vi "Configuration Tool Main.vi"() -> ()   [LabVIEW 2014, in "Advanced Configuration Tool.lvlib"]
doc: "This is the main VI for the configuration editor."
uses:
  Advanced Configuration Tool.lvlib
  Controls/StateCluster.ctl
  Configuration Framework/Repository/NISE_CEF_Repository.lvclass
  Configuration Framework/Node/NodeRef.ctl
  Configuration Framework/Node/NISE_CEF_Node.lvclass
  Configuration Framework/Node/StandardEvents.ctl
  Configuration Framework/Node/UserEventRef.ctl
  Configuration Framework/Controls/EventCluster.ctl
  Configuration Framework/Node/NodeChangeEvent.ctl
  Configuration Framework/Node/CacheState.ctl
  Configuration Framework/Node/RefreshUIEvent.ctl
  Configuration Framework/Node/StopEvent.ctl
  Configuration Framework/glyph manager/glyph manager.ctl
  <vilib>/picture/picture.llb/imagedata.ctl
  <vilib>/Utility/error.llb/DialogType.ctl
  Classes/cRIO node/cRIO  node root.lvclass
  Configuration Framework/hierarchy repo/NISE_CEF_HierarchyRepo.lvclass
  Controls/AddMessage.ctl
  Controls/MoveMessage.ctl
  <vilib>/NI/AMC/Read Termination Message.vi
  <vilib>/NI/AMC/Create Single Message.vi
  <vilib>/NI/AMC/Update Message Routing Info.vi
  <vilib>/NI/AMC/Globals.vi
  <vilib>/NI/AMC/Send Message.vi
  <vilib>/NI/AMC/AMC.lvlib
  Configuration Framework/NISE_CEF_TreeControl.lvlib
  Configuration Framework/serializable configuration/NISE_CEF_serializable configuration.lvclass
  Configuration Framework/glyph manager/glyph manager.lvlib
panel:
  in  "View":string(tree)
  in  "Exit":bool
  # "Configurator"
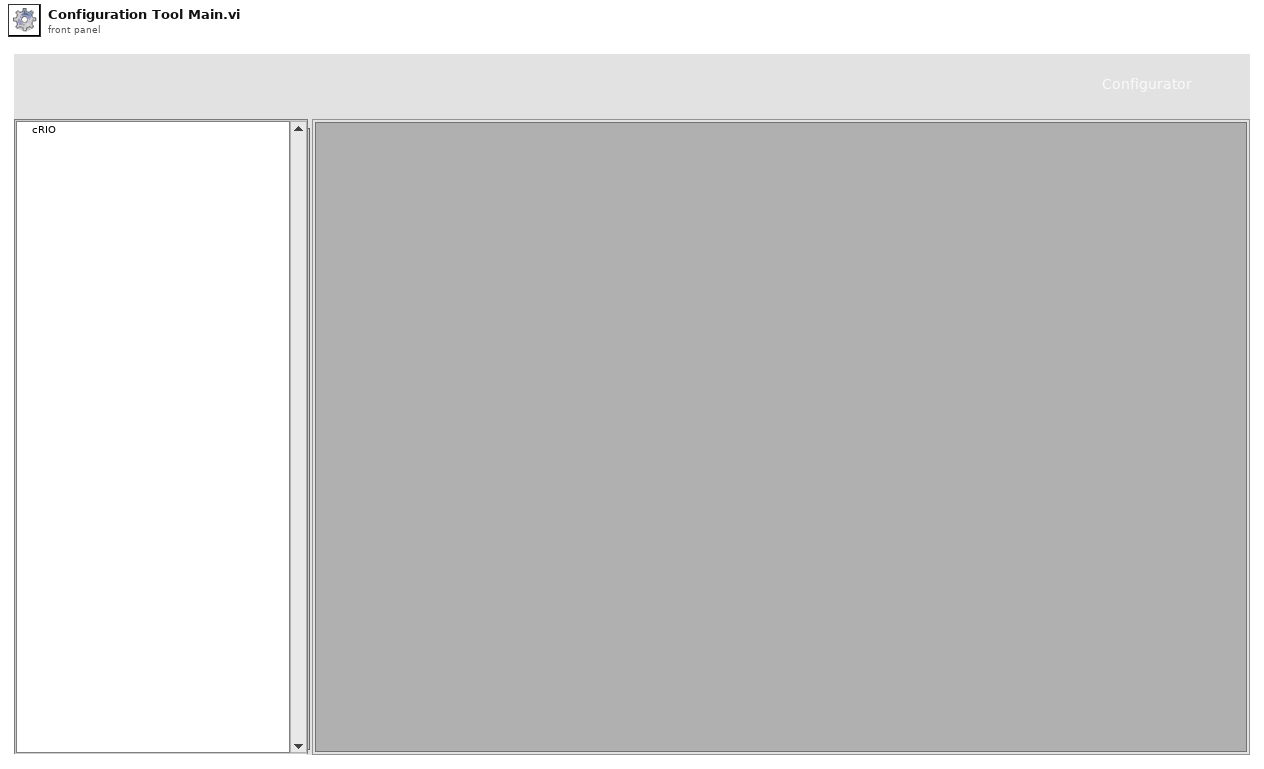
[diagram p1: front panel]
types:
  T1 = typedef "Advanced Configuration Tool.lvlib/StateCluster.ctl" = cluster{"repository":refnum<class "NISE_CEF_Repository.lvclass">, "root":T2, "unsaved changes":bool, "current path":path, "classes path":path, "standard events":T3, "glyph manager":T9}
  T2 = typedef "NISE_CEF_Node.lvclass/NodeRef.ctl" = refnum<data-value>
  T3 = typedef "NISE_CEF_Node.lvclass/StandardEvents.ctl" = cluster{"user event":T4, "node change":T5, "cache state":T6, "refresh UI":T7, "stop event":T8}
  T4 = typedef "NISE_CEF_Node.lvclass/UserEventRef.ctl" = refnum<user-event>
  T5 = typedef "NISE_CEF_Node.lvclass/NodeChangeEvent.ctl" = refnum<user-event>
  T6 = typedef "NISE_CEF_Node.lvclass/CacheState.ctl" = refnum<user-event>
  T7 = typedef "NISE_CEF_Node.lvclass/RefreshUIEvent.ctl" = refnum<user-event>
  T8 = typedef "NISE_CEF_Node.lvclass/StopEvent.ctl" = refnum<user-event>
  T9 = typedef "glyph manager.lvlib/glyph manager.ctl" = cluster{"search paths":path[], "glyph map":variant, "base glyphs":T10[], "desired overlays":string[]}
  T10 = typedef "imagedata.ctl" = cluster{"image type":i32, "image depth":i32, "image":u8[], "mask":u8[], "colors":u32[], "Rectangle":cluster{"left":i16, "top":i16, "right":i16, "bottom":i16}}
  T11 = typedef "AMC.lvlib/Message Queue.ctl" = refnum<queue>
  T12 = typedef "Advanced Configuration Tool.lvlib/AddMessage.ctl" = cluster{"node type":string, "to add to":string}
  T13 = typedef "Advanced Configuration Tool.lvlib/MoveMessage.ctl" = cluster{"node ref":T2, "new parent":T2, "Index":i32}
  T14 = typedef "Advanced Configuration Tool.lvlib/FilePaths.ctl" = cluster{"glyphs":path, "classes":path}
  T15 = typedef "DialogType.ctl" = u16
  T16 = typedef "NISE_CEF_Node.lvclass/Summary.ctl" = cluster{"ID":string, "parent ID":string, "node type":string, "text":string, "additional text":string, "glyph":string, "depth":i32, "glyph overlay":string}
  T17 = typedef "LVPoint32TypeDef.ctl" = cluster{"Horizontal":i32, "Vertical":i32}
  T18 = cluster{"data name":string, "drag data":variant}[]
  T19 = typedef "NISE_CEF_Node.lvclass/NodeMenuOptions.ctl" = cluster{"removable":bool, "movable":bool, "duplicate":bool}
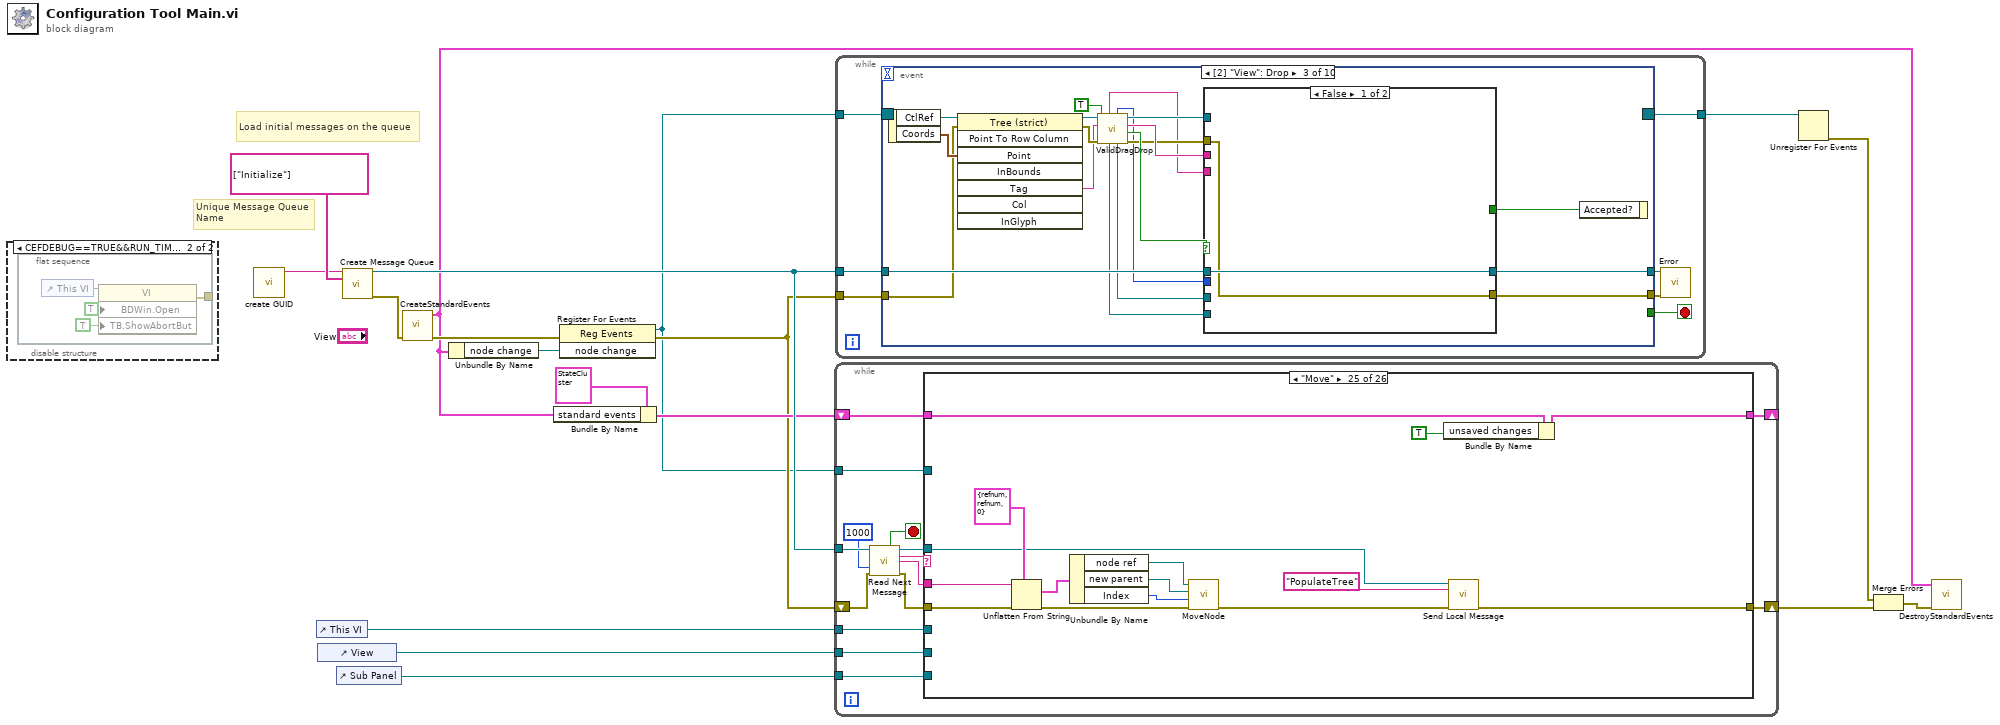
[diagram p0: block diagram]
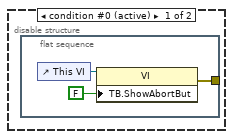
[diagram p2: hidden frame]
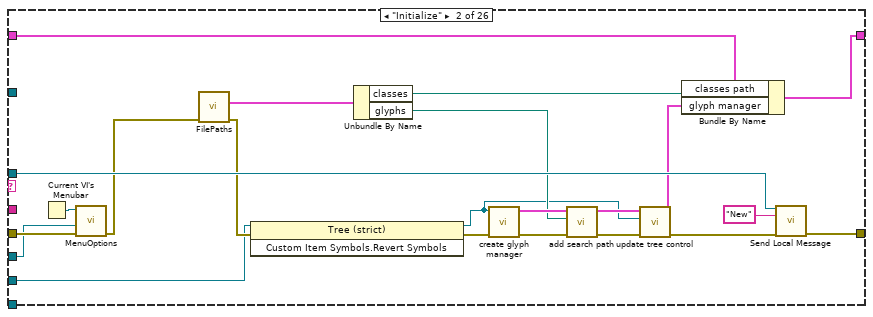
[diagram p4: hidden frame]
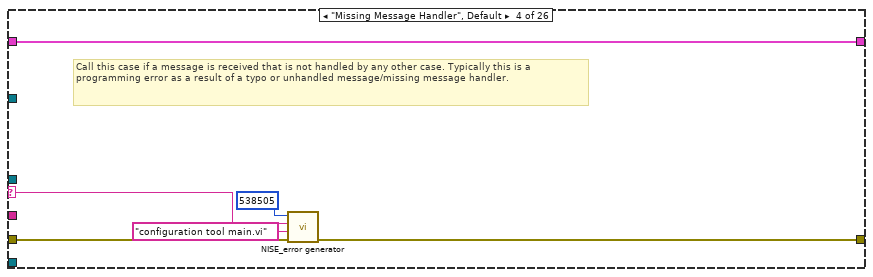
[diagram p6: hidden frame]
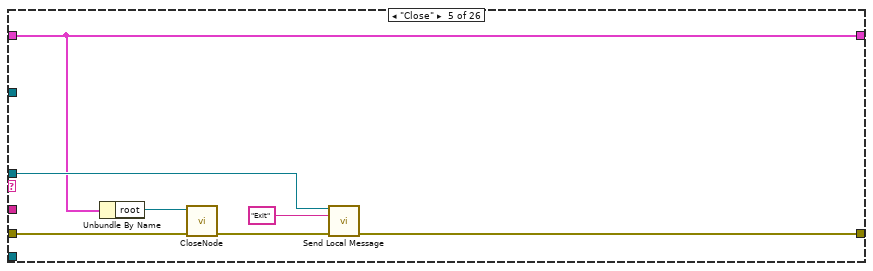
[diagram p7: hidden frame]
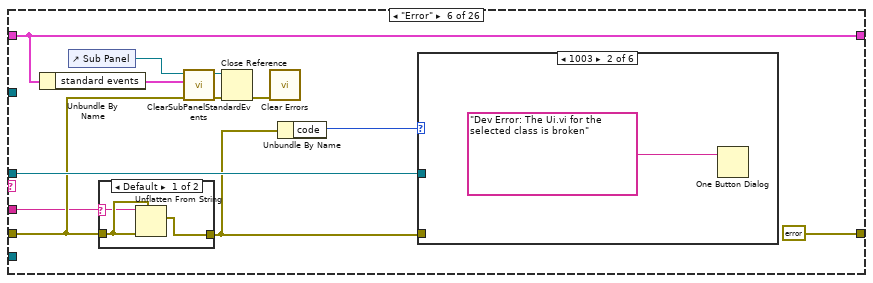
[diagram p8: hidden frame]
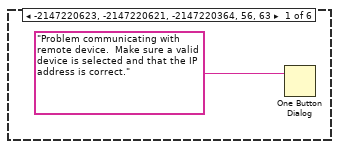
[diagram p10: hidden frame]
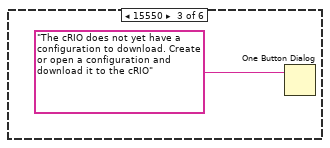
[diagram p11: hidden frame]
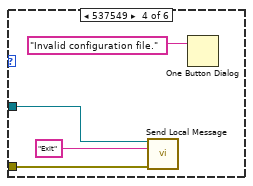
[diagram p12: hidden frame]
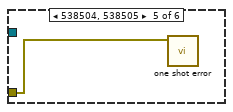
[diagram p13: hidden frame]
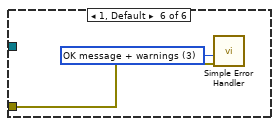
[diagram p14: hidden frame]
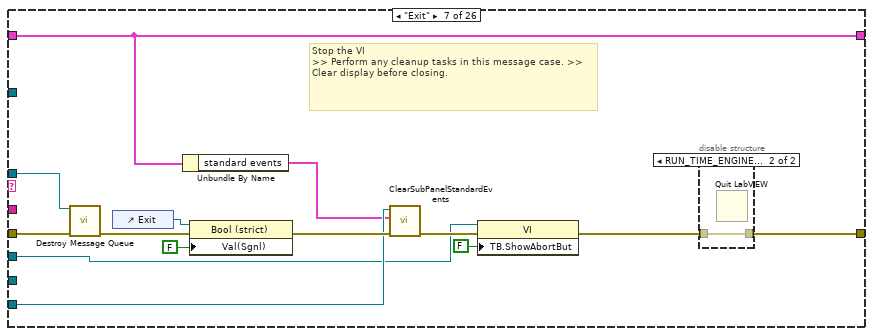
[diagram p15: hidden frame]
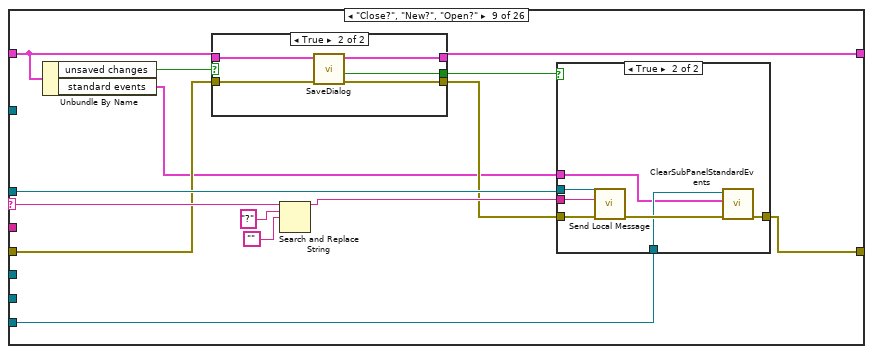
[diagram p18: hidden frame]
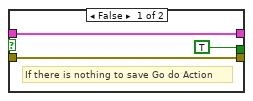
[diagram p19: hidden frame]
diagram:
  # "Unique Message Queue Name"
  # "Load initial messages on the queue"
  n1 = disable-structure shown="CEFDEBUG==TRUE&&RUN_TIME_ENGINE==False" {
    frame condition #0 (active) {
      n2 = flat-sequence {
        tunnel: [w19] -> _
        frame #0 {
          n3 = control-ref of="This VI"() -> (w20:refnum<vi>)
          n4 = property class="VI"(reference=w20, "TB.ShowAbortBut"=FALSE ("Tool Bar:Show Abort Button")) -> (error out=w19:errorcluster)  [unwired: 1 in, 1 out]
        }
      }
    }
    frame condition #1 {
      n5 = flat-sequence {
        tunnel: [w24] -> _
        frame #0 {
          n6 = control-ref of="This VI"() -> (w25:refnum<vi>)
          n7 = property class="VI"(reference=w25, "BDWin.Open"=TRUE ("Block Diagram Window:Open"), "TB.ShowAbortBut"=TRUE ("Tool Bar:Show Abort Button")) -> (error out=w24:errorcluster)  [unwired: 1 in, 1 out]
        }
      }
    }
  }
  n8 = call "create GUID.vi"() -> ("uuid"=w12:string)  [unwired: 10 in, 1 out]
  n9 = control-ref of="This VI"() -> (w15:refnum<vi>)
  n10 = control-ref of="View"() -> (w14:refnum<vi>)
  n11 = control-ref of="Sub Panel"() -> (w13:refnum<vi>)
  n12 = call <vilib>:"Create Message Queue.vi"("message queue name"=w12, "initial message names"=string[] ["Initialize"]) -> ("message queue out"=w17:T11, "error out"=w10:errorcluster)  [unwired: 12 in]
  n13 = call "CreateStandardEvents.vi"("error in"=w10) -> ("error out"=w9:errorcluster, "standard events"=w4:T3)  [unwired: 9 in]
  n14 = Unbundle By Name(w4) -> ("node change"=w7:T5)
  n15 = Bundle By Name(cluster=T1 {"repository"=refnum, "root"=refnum, "unsaved changes"=FALSE, "current path"=path "", "classes path"=path "", "standard events"={"user event"=refnum, "node change"=refnum, "cache state"=refnum, "refresh UI"=refnum, "stop event"=refnum}, "glyph manager"={"search paths"=[], "glyph map"=variant, "base glyphs"=[], "desired overlays"=[]}}, "standard events"=w4) -> (w11:T1)
  n16 = register-events(error in=w9, w7) -> (reference out=w5:refnum<event-registration>, error out=w8:errorcluster)  [unwired: 1 in]
  n17 = while "Message Processor" {
    shift-right: [w36] -> w1
    shift-left: w8 -> [w35]
    tunnel: w17 -> [w34]
    shift-right: [w32] -> _
    shift-left: w11 -> [w31]
    tunnel: w15 -> [w29]
    tunnel: w14 -> [w28]
    tunnel: w13 -> [w27]
    tunnel: w5 -> [w26]
    stop <- w40 stop-if-true
    n18 = call <vilib>:"Read Next Message.vi"("message queue in"=w34, "timeout (1 ms)"=1000, "error in"=w35) -> ("exit process?"=w40:bool, "message queue out"=w30:T11, "message name"=w39:string, "message value"=w38:string, "error out"=w37:errorcluster)  [unwired: 5 in, 3 out]
    n19 = case shown="\"Move\"" w39 {
      selector: w39 -> [_ _ _ w69 _ _ _ _ w133 _ _ _ _ _ _ _ _ _ w373 _ _ _ _ _ _ _]
      tunnel: w38 -> [_ _ _ _ _ w81 _ _ _ _ _ _ _ w256 w288 _ w331 w348 w371 w430 w456 _ _ w503 w526 w529]
      tunnel: w37 -> [w42 w64 w66 w71 w74 w84 w119 w123 w126 w164 w176 w220 w249 w263 w289 w306 w308 w347 w376 w432 w455 w484 w493 w502 w524 w531]
      tunnel: [w42 w61 w66 w70 w78 errorcluster {"status"=FALSE, "code"=0, "source"=""} ("error out") w112 w123 w137 w156 w172 w223 w246 w260 w276 w306 w325 w351 w379 w434 w452 w479 w489 w499 w519 w530] -> w36
      tunnel: [w41 w57 w65 w72 w76 w88 w111 w122 w128 w169 w177 w226 w250 w257 w285 w305 w318 w344 w367 w433 w449 w468 w492 w497 w515 w534] -> w32
      tunnel: w31 -> [w41 w58 w65 w72 w76 w88 w111 w122 w129 w167 w178 w217 w248 w258 w286 w305 w322 w342 w367 w425 w457 w486 w492 w497 w527 w535]
      tunnel: w30 -> [_ w60 _ _ w77 w91 w118 _ w136 w170 w174 w222 _ w259 w281 _ _ _ w374 _ _ _ _ w498 w518 w528]
      tunnel: w29 -> [_ w55 _ _ _ _ w108 _ _ _ _ _ _ _ _ _ _ _ _ _ _ w472 _ _ _ _]
      tunnel: w28 -> [_ w44 _ _ _ _ _ _ _ _ _ _ _ _ _ _ w319 w345 w368 w427 w450 w473 _ _ _ _]
      tunnel: w27 -> [_ _ _ _ _ _ w110 _ w124 _ _ _ _ _ _ _ _ _ _ _ _ w470 w488 w494 _ _]
      tunnel: w26 -> [_ _ _ _ _ _ _ _ _ _ _ w216 w247 _ _ _ _ _ _ _ _ _ _ _ _ _]
      frame "------------Generic Operations------------" {
        # "Dummy case to add a seperation in the Case Structure menu"
      }
      frame "Initialize" {
        n20 = Current VI's Menubar() -> (w63:refnum<k9>)
        n21 = call "MenuOptions.vi"("error in"=w64, "VI ref"=w55, "menu ref in"=w63) -> ("error out"=w54:errorcluster)  [unwired: 7 in, 1 out]
        n22 = call "FilePaths.vi"("error in"=w54) -> ("error out"=w53:errorcluster, "paths"=w59:T14)  [unwired: 9 in]
        n23 = invoke class="Tree (strict)" method="Custom Item Symbols.Revert Symbols"(reference=w44, error in=w53) -> (reference out=w43:refnum<vi>, error out=w45:errorcluster)  [unwired: 1 in, 1 out]
        n24 = Unbundle By Name(w59) -> ("classes"=w56:path, "glyphs"=w50:path)
        n25 = call "create glyph manager.vi"("error in"=w45, "tree ref (for default symbols)"=w43) -> ("error out"=w52:errorcluster, "glyph manager"=w51:T9)  [unwired: 8 in]
        n26 = call "add search path.vi"("error in"=w52, "search path"=w50, "glyph manager in"=w51) -> ("error out"=w49:errorcluster, "glyph manager out"=w47:T9)  [unwired: 7 in]
        n27 = call "update tree control.vi"("error in"=w49, "tree reference"=w43, "glyph manager in"=w47) -> ("error out"=w48:errorcluster, "glyph manager out"=w46:T9)  [unwired: 7 in]
        n28 = Bundle By Name(cluster=w58, "classes path"=w56, "glyph manager"=w46) -> (w57:T1)
        n29 = call <vilib>:"Send Local Message.vi"("message queue in"=w60, "message name"="New" ("Message Name"), "error in"=w48) -> ("error out"=w61:errorcluster)  [unwired: 10 in, 2 out]
      }
      frame "", "Idle" {
      }
      frame "Missing Message Handler", Default {
        # "Call this case if a message is received that is not handled by any other case. Typically this is a programming error as a result of a typo or unhandled message/missing message handler."
        n30 = call "NISE_error generator.vi"("error in"=w71, "source"="configuration tool main.vi", "append error message"=w69, "error code (0)"=538505) -> ("error out"=w70:errorcluster)  [unwired: 5 in]
      }
      frame "Close" {
        n31 = Unbundle By Name(w76) -> ("root"=w75:T2)
        n32 = call "CloseNode.vi"("error in"=w74, "node ref"=w75) -> ("error out"=w73:errorcluster)  [unwired: 9 in]
        n33 = call <vilib>:"Send Local Message.vi"("message queue in"=w77, "message name"="Exit", "error in"=w73) -> ("error out"=w78:errorcluster)  [unwired: 10 in, 2 out]
      }
      frame "Error" {
        n34 = Unbundle By Name(w88) -> ("standard events"=w80:T3)
        n35 = control-ref of="Sub Panel"() -> (w87:refnum<vi>)
        n36 = case shown="Default" w81 {
          selector: w81 -> [w93 _]
          tunnel: w84 -> [w94 w95]
          tunnel: [w92 w95] -> w83
          frame Default {
            n37 = Unflatten From String(type=w94, binary string=w93, error in (no error)=w94) -> (value=w92:errorcluster)  [unwired: 2 in, 2 out]
          }
          frame "" {
          }
        }
        n38 = call "ClearSubPanelStandardEvents.vi"("error in"=w84, "standard events"=w80, "sub panel ref in"=w87) -> ("error out"=w86:errorcluster, "sub panel ref out"=w85:refnum<vi>)  [unwired: 7 in]
        n39 = Close Reference(reference=w85, error in (no error)=w86) -> (error out=w82:errorcluster)
        n40 = call <vilib>:"Clear Errors.vi"("error in (no error)"=w82) -> ()  [unwired: 5 in, 2 out]
        n41 = Unbundle By Name(w83) -> ("code"=w89:i32)
        n42 = case shown="1003" w89 {
          tunnel: w91 -> [_ _ _ w101 _ _]
          tunnel: w83 -> [_ _ _ w100 w103 w105]
          frame -2147220623, -2147220621, -2147220364, 56, 63 {
            n43 = One Button Dialog(message="Problem communicating with remote device.  Make sure a valid device is selected and that the IP address is correct.") -> ()  [unwired: 1 in, 1 out]
          }
          frame 1003 {
            n44 = One Button Dialog(message="Dev Error: The Ui.vi for the selected class is broken") -> ()  [unwired: 1 in, 1 out]
          }
          frame 15550 {
            n45 = One Button Dialog(message="The cRIO does not yet have a configuration to download. Create or open a configuration and download it to the cRIO") -> ()  [unwired: 1 in, 1 out]
          }
          frame 537549 {
            n46 = call <vilib>:"Send Local Message.vi"("message queue in"=w101, "message name"="Exit", "error in"=w100) -> ()  [unwired: 10 in, 3 out]
            n47 = One Button Dialog(message="Invalid configuration file.") -> ()  [unwired: 1 in, 1 out]
          }
          frame 538504, 538505 {
            n48 = call "one shot error.vi"("error in"=w103) -> ()  [unwired: 11 in]
          }
          frame 1, Default {
            w104 = T15 3 items=["no dialog", "OK message", "continue or stop message", "OK message + warnings", "continue/stop + warnings"] ("type of dialog (OK msg:1)")
            n49 = call <vilib>:"Simple Error Handler.vi"("type of dialog (OK msg:1)"=w104, "error in (no error)"=w105) -> ()  [unwired: 8 out]
          }
        }
      }
      frame "Exit" {
        # "Stop the VI                                                                             >> Perform any cleanup tasks in this message case. >> Clear display before closing."
        n50 = call <vilib>:"Destroy Message Queue.vi"("message queue in"=w118, "error in"=w119) -> ("error out"=w115:errorcluster)  [unwired: 11 in, 2 out]
        n51 = control-ref of="Exit"() -> (w117:refnum<vi>)
        n52 = Unbundle By Name(w111) -> ("standard events"=w106:T3)
        n53 = property class="Bool (strict)"(reference=w117, error in=w115, "Val(Sgnl)"=FALSE ("Exit")) -> (error out=w114:errorcluster)  [unwired: 1 out]
        n54 = call "ClearSubPanelStandardEvents.vi"("error in"=w114, "standard events"=w106, "sub panel ref in"=w110) -> ("error out"=w113:errorcluster)  [unwired: 7 in, 1 out]
        n55 = property class="VI"(reference=w108, error in=w113, "TB.ShowAbortBut"=FALSE ("Tool Bar:Show Abort Button")) -> (error out=w109:errorcluster)  [unwired: 1 out]
        n56 = disable-structure shown="RUN_TIME_ENGINE==True" {
          disable-tunnel: [w120 w121] -> w112
          disable-tunnel: w109 -> [w120 w121]
          frame condition #0 (active) {
          }
          frame condition #1 {
            n57 = Quit LabVIEW() -> ()  [unwired: 1 in]
          }
        }
      }
      frame "------------Menu Operations--------------" {
        # "Dummy case to add a seperation in the Case Structure menu"
      }
      frame "Close?", "New?", "Open?" {
        n58 = Unbundle By Name(w129) -> ("unsaved changes"=w131:bool, "standard events"=w125:T3)
        n59 = case shown="True" w131 {
          tunnel: [TRUE ("SaveFlag") w145] -> w130
          tunnel: w129 -> [w139 w144]
          tunnel: [w139 w143] -> w128
          tunnel: w126 -> [w138 w142]
          tunnel: [w138 w141] -> w127
          frame False {
            # "If there is nothing to save Go do Action"
          }
          frame True {
            n60 = call "SaveDialog.vi"("error in"=w142, "state in"=w144) -> ("error out"=w141:errorcluster, "new"=w145:bool, "state out"=w143:T1)  [unwired: 7 in]
          }
        }
        n61 = Search and Replace String(input string=w133, search string="?", replace string="") -> (result string=w132:string)  [unwired: 5 in, 3 out]
        n62 = case shown="True" w130 {
          tunnel: w127 -> [w146 w153]
          tunnel: [w146 w149] -> w137
          tunnel: w136 -> [_ w152]
          tunnel: w132 -> [_ w151]
          tunnel: w125 -> [_ w147]
          tunnel: w124 -> [_ w148]
          frame False {
          }
          frame True {
            n63 = call <vilib>:"Send Local Message.vi"("message queue in"=w152, "message name"=w151, "error in"=w153) -> ("error out"=w150:errorcluster)  [unwired: 10 in, 2 out]
            n64 = call "ClearSubPanelStandardEvents.vi"("error in"=w150, "standard events"=w147, "sub panel ref in"=w148) -> ("error out"=w149:errorcluster)  [unwired: 7 in, 1 out]
          }
        }
      }
      frame "New" {
        n65 = Unbundle By Name(w167) -> ("classes path"=w166:path)
        n66 = call-dynamic "Initialize.vi"("error in"=w164, "path"=w166, "repository in"=refnum<class "NISE_CEF_HierarchyRepo.lvclass"> refnum ("NISE_CEF_HierarchyRepo.lvclass")) -> ("error out"=w154:errorcluster, "repository out"=w158:refnum<class "NISE_CEF_HierarchyRepo.lvclass">)  [unwired: 7 in]
        n67 = call-dynamic "Initialize.vi"("error in"=w154, "cRIO in"=refnum<class "cRIO  node root.lvclass"> refnum ("_cRIO.lvclass")) -> ("error out"=w165:errorcluster, "data value reference"=w168:T2)  [unwired: 7 in, 1 out]
        n68 = call <vilib>:"Send Local Message.vi"("message queue in"=w170, "message name"="PopulateTree", "error in"=w165) -> ("error out"=w160:errorcluster)  [unwired: 10 in, 2 out]
        n69 = Current VI's Menubar() -> (w159:refnum<k9>)
        n70 = call "NewMenu.vi"("error in"=w160, "menu ref in"=w159, "NISE_CEF_Repository in"=w158) -> ("error out"=w156:errorcluster, "NISE_CEF_Repository out"=w157:refnum<class "NISE_CEF_HierarchyRepo.lvclass">)  [unwired: 6 in, 1 out]
        n71 = Bundle By Name(cluster=w167, "current path"=path "", "unsaved changes"=FALSE, "repository"=w157, "root"=w168) -> (w169:T1)
      }
      frame "Open" {
        n72 = in-place {
          in-place-border: w176 -> [w184]
          in-place-border: [w183] -> w173
          n73 = in-place-cluster #1(w178) -> ("current path"=w180:path, "repository"=w192:refnum<class "NISE_CEF_Repository.lvclass">, "root"=w188:T2)  [unwired: 1 out]
          n74 = call "generate default path.vi"("current file path"=w180) -> ("browse path"=w179:path)  [unwired: 10 in]
          n75 = call "FileDialog.vi"("error in"=w184, "start path"=w179) -> ("error out"=w185:errorcluster, "cancelled"=w186:bool, "selected path"=w182:path)  [unwired: 7 in]
          n76 = Compound Arithmetic op=OR(invert w186) -> (w187:bool)
          n77 = case shown="True" w187 {
            tunnel: w192 -> [w193 w205]
            tunnel: [w193 w203] -> w190
            tunnel: [w194 w201] -> w183
            tunnel: [w195 w200] -> w189
            tunnel: w182 -> [_ w198]
            tunnel: w185 -> [w194 w197]
            tunnel: w188 -> [w195 w196]
            frame False {
            }
            frame True {
              n78 = call-dynamic "Open.vi"("error in"=w197, "file path"=w198, "repository in"=w205) -> ("error out"=w202:errorcluster, "invalid?"=w199:bool, "repository out"=w204:refnum<class "NISE_CEF_Repository.lvclass">)  [unwired: 6 in]
              n79 = case shown="False" w199 {
                tunnel: w204 -> [w210 w213]
                tunnel: [w209 w213] -> w203
                tunnel: w202 -> [w208 w212]
                tunnel: [w207 w212] -> w201
                tunnel: [w206 w211] -> w200
                tunnel: w196 -> [_ w211]
                frame False {
                  n80 = call-dynamic "WriteTree.vi"("error in"=w208, "repository in"=w210) -> ("error out"=w207:errorcluster, "root"=w206:T2, "repository out"=w209:refnum<class "NISE_CEF_Repository.lvclass">)  [unwired: 7 in]
                }
                frame True {
                }
              }
            }
          }
          n81 = Select(t=w180, s=w183, f=w182) -> (s? t:f=w181:path)
          n82 = in-place-cluster #1("current path"=w181, "unsaved changes"=FALSE ("SaveFlag"), "repository"=w190, "root"=w189) -> (w177:T1)
        }
        n83 = call <vilib>:"Send Local Message.vi"("message queue in"=w174, "message name"="PopulateTree", "error in"=w173) -> ("error out"=w172:errorcluster)  [unwired: 10 in, 2 out]
      }
      frame "Save" {
        n84 = in-place {
          in-place-border: w220 -> [w231]
          in-place-border: [w230] -> w215
          in-place-border: [w228] -> w219
          n85 = in-place-cluster #2(w217) -> ("current path"=w229:path, "root"=w232:T2, "repository"=w233:refnum<class "NISE_CEF_Repository.lvclass">)
          n86 = Empty String/Path?(string/path=w229) -> (empty?=w228:bool)
          n87 = call-dynamic "ReadTree.vi"("error in"=w231, "root"=w232, "repository in"=w233) -> ("error out"=w230:errorcluster, "repository out"=w227:refnum<class "NISE_CEF_Repository.lvclass">)  [unwired: 7 in]
          n88 = in-place-cluster #2("current path"=w229, "root"=w232, "repository"=w227) -> (w221:T1)
        }
        n89 = Unbundle By Name(w217) -> ("standard events.node change"=w218:T5)
        n90 = Flush Event Queue(0:w216, 2:w218, 3:w215) -> (11:w214:errorcluster)  [unwired: 3 in, 2 out]
        n91 = case shown="True" w219 {
          tunnel: w221 -> [w237 w239]
          tunnel: [w236 w238] -> w226
          tunnel: [w235 w240] -> w224
          tunnel: w214 -> [w234 w241]
          frame False {
            n92 = call "Save.vi"("error in"=w234, "state in"=w237) -> ("error out"=w235:errorcluster, "state out"=w236:T1)  [unwired: 8 in]
          }
          frame True {
            # "Empty path use Dialog"
            n93 = call "SaveAs.vi"("error in"=w241, "state in"=w239) -> ("error out"=w240:errorcluster, "state out"=w238:T1)  [unwired: 7 in, 1 out]
          }
        }
        n94 = call <vilib>:"Send Local Message.vi"("message queue in"=w222, "message name"="PopulateTree", "error in"=w224) -> ("error out"=w223:errorcluster)  [unwired: 10 in, 2 out]
      }
      frame "SaveAs" {
        n95 = in-place {
          in-place-border: w249 -> [w252]
          in-place-border: [w251] -> w245
          n96 = in-place-cluster #3(w248) -> ("root"=w253:T2, "repository"=w255:refnum<class "NISE_CEF_Repository.lvclass">)
          n97 = call-dynamic "ReadTree.vi"("error in"=w252, "root"=w253, "repository in"=w255) -> ("error out"=w251:errorcluster, "repository out"=w254:refnum<class "NISE_CEF_Repository.lvclass">)  [unwired: 7 in]
          n98 = in-place-cluster #3("root"=w253, "repository"=w254) -> (w243:T1)
        }
        n99 = Unbundle By Name(w243) -> ("standard events.node change"=w242:T5)
        n100 = Flush Event Queue(0:w247, 2:w242, 3:w245) -> (11:w244:errorcluster)  [unwired: 3 in, 2 out]
        n101 = call "SaveAs.vi"("error in"=w244, "state in"=w243) -> ("error out"=w246:errorcluster, "state out"=w250:T1)  [unwired: 7 in, 1 out]
      }
      frame "Custom View" {
        n102 = in-place {
          in-place-border: w263 -> [w274]
          in-place-border: [w273] -> w261
          in-place-border: w256 -> [w264]
          n103 = in-place-cluster #4(w258) -> ("repository"=w268:refnum<class "NISE_CEF_Repository.lvclass">, "root"=w267:T2)
          n104 = call-dynamic "ReadTree.vi"("error in"=w274, "root"=w267, "repository in"=w268) -> ("error out"=w271:errorcluster, "repository out"=w270:refnum<class "NISE_CEF_Repository.lvclass">)  [unwired: 7 in]
          n105 = call-dynamic "CustomView.vi"("error in"=w271, "view name"=w264, "repository in"=w270) -> ("error out"=w272:errorcluster, "repository out"=w269:refnum<class "NISE_CEF_Repository.lvclass">)  [unwired: 7 in]
          n106 = call-dynamic "WriteTree.vi"("error in"=w272, "repository in"=w269) -> ("error out"=w273:errorcluster, "root"=w265:T2, "repository out"=w266:refnum<class "NISE_CEF_Repository.lvclass">)  [unwired: 7 in]
          n107 = in-place-cluster #4("repository"=w266, "root"=w265) -> (w257:T1)
        }
        n108 = call <vilib>:"Send Local Message.vi"("message queue in"=w259, "message name"="PopulateTree", "error in"=w261) -> ("error out"=w260:errorcluster)  [unwired: 10 in, 2 out]
      }
      frame "CustomFileMenu" {
        n109 = Unflatten From String(type=cluster{"ItemTag":string, string} {"ItemTag"="", ""} ("output cluster"), binary string=w288, error in (no error)=w289) -> (value=w275:cluster{"ItemTag":string, string}, error out=w284:errorcluster)  [unwired: 2 in, 1 out]
        n110 = Unbundle By Name(w286) -> ("repository"=w283:refnum<class "NISE_CEF_Repository.lvclass">)
        n111 = Unbundle(w275) -> ("ItemTag"=w280:string, w279:string)
        n112 = call-dynamic "HandleMenu.vi"("message queue"=w281, "error in"=w284, "Item Path"=w279, "ItemTag"=w280, "NISE_CEF_Repository in"=w283) -> ("error out"=w278:errorcluster, "handled?"=w277:bool, "NISE_CEF_Repository out"=w282:refnum<class "NISE_CEF_Repository.lvclass">)  [unwired: 4 in]
        n113 = case shown="True" w277 {
          tunnel: w278 -> [w293 w304]
          tunnel: [w294 w304] -> w276
          tunnel: w275 -> [w292 _]
          frame False {
            n114 = Unbundle(w292) -> ("ItemTag"=w291:string, w290:string)
            n115 = disable-structure shown="Default" {
              disable-tunnel: w293 -> [w300 w303]
              disable-tunnel: [w299 w303] -> w294
              disable-tunnel: w290 -> [w298 _]
              disable-tunnel: w291 -> [w297 _]
              frame condition #0 {
                n116 = Concatenate Strings(w297, "::" ("string"), w298) -> (w296:string)
                n117 = call "NISE_error generator.vi"("error in"=w300, "source"="configuration tool main.vi", "append error message"=w296, "error code (0)"=538506) -> ("error out"=w299:errorcluster)  [unwired: 5 in]
              }
              frame condition #1 (active) {
              }
            }
          }
          frame True {
          }
        }
        n118 = Bundle By Name(cluster=w286, "repository"=w282) -> (w285:T1)
      }
      frame "-------TreeControl Operations-----------" {
        # "Dummy case to add a seperation in the Case Structure menu"
      }
      frame "AddNode" {
        n119 = Unflatten From String(type=T12 {"node type"="", "to add to"=""} ("input cluster"), binary string=w331, error in (no error)=w308) -> (value=w329:T12, error out=w307:errorcluster)  [unwired: 2 in, 1 out]
        n120 = Unbundle By Name(w329) -> ("to add to"=w327:string, "node type"=w321:string)
        n121 = in-place {
          in-place-border: w307 -> [w337]
          in-place-border: [w336] -> w323
          in-place-border: w321 -> [w335]
          in-place-border: [w334] -> w320
          n122 = in-place-cluster #5(w322) -> ("repository"=w339:refnum<class "NISE_CEF_Repository.lvclass">)
          n123 = call-dynamic "GetClassPath.vi"("error in"=w337, "class name"=w335, "Repository in"=w339) -> ("error out"=w336:errorcluster, "class path"=w334:path, "Repository out"=w338:refnum<class "NISE_CEF_Repository.lvclass">)  [unwired: 6 in]
          n124 = in-place-cluster #5("repository"=w338) -> (w316:T1)
        }
        n125 = Unbundle By Name(w316) -> ("glyph manager"=w313:T9)
        n126 = call <vilib>:"Get LV Class Default Value.vi"("error in (no error)"=w323, "class path"=w320) -> ("error out"=w332:errorcluster, "object"=w333:refnum<class>)  [unwired: 8 in]
        n127 = To More Specific Class(target class=refnum<class "NISE_CEF_Node.lvclass"> refnum ("Node.lvclass"), reference=w333, error in=w332) -> (specific class reference=w314:refnum<class "NISE_CEF_Node.lvclass">, error out=w315:errorcluster)
        n128 = call-dynamic "AddGlyphtoGManager.vi"("error in"=w315, "glyph manager"=w313, "NISE_CEF_Node in"=w314) -> ("error out"=w312:errorcluster, "glyph manager out"=w310:T9, "NISE_CEF_Node out"=w311:refnum<class "NISE_CEF_Node.lvclass">)  [unwired: 6 in]
        n129 = call "AddNode.vi"("error in"=w312, "node in"=w311, "parent node ID"=w327) -> ("error out"=w326:errorcluster, "summary"=w324:T16[])  [unwired: 7 in]
        n130 = call "PopulateTreeSumaryWithGlyphManager.vi"("error in"=w326, "glyph manager"=w310, "summary"=w324, "tree ref in"=w319) -> ("error out"=w325:errorcluster, "glyph manager out"=w309:T9)  [unwired: 6 in]
        n131 = Bundle By Name(cluster=w316, "unsaved changes"=TRUE, "glyph manager"=w309) -> (w318:T1)
      }
      frame "Duplicate" {
        n132 = Unbundle By Name(w342) -> ("glyph manager"=w341:T9)
        n133 = call "IDtoNode.vi"("error in"=w347, "ID"=w348) -> ("error out"=w349:errorcluster, "invalid Id"=w346:bool, "node ref"=w350:T2)  [unwired: 7 in]
        n134 = case shown="False" w346 {
          tunnel: [w363 w365] -> w351
          tunnel: w350 -> [w362 _]
          tunnel: w349 -> [w359 w365]
          tunnel: w345 -> [w355 _]
          tunnel: w341 -> [w352 w364]
          tunnel: [w354 w364] -> w340
          frame False {
            n135 = call "DuplicateNode.vi"("same parent?"=TRUE ("s"), "error in"=w359, "node ref in"=w362) -> ("error out"=w360:errorcluster, "new node ref"=w361:T2)  [unwired: 7 in]
            n136 = call "SummaryWithGlyphManager.vi"("error in"=w360, "glyph manager"=w352, "node self ref"=w361) -> ("error out"=w357:errorcluster, "glyph manager out"=w353:T9, "summary"=w356:T16[])  [unwired: 6 in]
            n137 = call "PopulateTreeSumaryWithGlyphManager.vi"("error in"=w357, "glyph manager"=w353, "summary"=w356, "tree ref in"=w355) -> ("error out"=w363:errorcluster, "glyph manager out"=w354:T9)  [unwired: 6 in]
          }
          frame True {
          }
        }
        n138 = Bundle By Name(cluster=w342, "unsaved changes"=TRUE, "glyph manager"=w340) -> (w344:T1)
      }
      frame "CustomMenuAction" {
        n139 = Match Pattern(string=w371, regular expression=":") -> (before substring=w370:string, after substring=w369:string)  [unwired: 1 in, 2 out]
        n140 = Unbundle By Name(w367) -> ("standard events.node change"=w366:T5)
        n141 = call "IDtoNode.vi"("error in"=w376, "ID"=w369) -> ("error out"=w377:errorcluster, "invalid Id"=w375:bool, "node ref"=w378:T2)  [unwired: 7 in]
        n142 = case shown="False" w375 {
          tunnel: [w388 w423] -> w379
          tunnel: w378 -> [w385 _]
          tunnel: w377 -> [w391 w423]
          tunnel: w374 -> [w392 _]
          tunnel: w373 -> [_ _]
          tunnel: w370 -> [w389 _]
          tunnel: w368 -> [w386 _]
          tunnel: w366 -> [w382 _]
          frame False {
            n143 = in-place {
              in-place-border: w392 -> [w421]
              in-place-border: w391 -> [w419]
              in-place-border: [w418] -> w387
              in-place-border: [w417] -> w390
              in-place-border: w389 -> [w416]
              in-place-border: w386 -> [w415]
              in-place-border: [w412] -> w381
              n144 = in-place-dvr #6(w385) -> (w422:refnum<class "NISE_CEF_Node.lvclass">, w413:errorcluster)
              n145 = Merge Errors(w413, w419) -> (w414:errorcluster)
              n146 = call-dynamic "MenuHandler.vi"("tree control"=w415, "main message queue"=w421, "error in"=w414, "menu string"=w416, "NISE_CEF_Node in"=w422) -> ("error out"=w418:errorcluster, "refresh tree?"=w412:bool, "Unhandled"=w417:bool, "NISE_CEF_Node out"=w420:refnum<class "NISE_CEF_Node.lvclass">)  [unwired: 3 in]
              n147 = in-place-dvr #6(w420) -> (w380:T2, w383:errorcluster)
            }
            n148 = Merge Errors(w383, w387) -> (w384:errorcluster)
            n149 = case shown="False" w390 {
              tunnel: w389 -> [_ w403]
              tunnel: [w396 w404] -> w388
              tunnel: w384 -> [w397 w405]
              tunnel: w382 -> [w395 _]
              tunnel: w381 -> [w394 _]
              tunnel: w380 -> [w393 _]
              frame False {
                n150 = case shown="False" w394 {
                  tunnel: w397 -> [w398 w402]
                  tunnel: [w398 w401] -> w396
                  tunnel: w395 -> [_ w400]
                  tunnel: w393 -> [_ w399]
                  frame False {
                  }
                  frame True {
                    n151 = Generate User Event(user event=w400, event data cluster=w399, error in=w402) -> (error out=w401:errorcluster)  [unwired: 1 in, 1 out]
                  }
                }
              }
              frame True {
                n152 = disable-structure shown="CEFDEBUG==TRUE" {
                  disable-tunnel: w405 -> [w408 w411]
                  disable-tunnel: [w407 w411] -> w404
                  disable-tunnel: w403 -> [w406 _]
                  frame condition #0 {
                    n153 = call "NISE_error generator.vi"("error in"=w408, "source"="configuration tool main.vi", "append error message"=w406, "error code (0)"=538506) -> ("error out"=w407:errorcluster)  [unwired: 5 in]
                  }
                  frame condition #1 (active) {
                  }
                }
              }
            }
          }
          frame True {
          }
        }
      }
      frame "RefreshNode" {
        # "Refreshes the node in the Tree, Sets the save flag to true. This case can be called from the UIs of the nodes"
        n154 = Unbundle By Name(w425) -> ("glyph manager"=w424:T9)
        n155 = call "IDtoNode.vi"("error in"=w432, "ID"=w430) -> ("error out"=w431:errorcluster, "invalid Id"=w428:bool, "node ref"=w429:T2)  [unwired: 7 in]
        n156 = case shown="False" w428 {
          tunnel: [w444 w447] -> w434
          tunnel: w431 -> [w440 w447]
          tunnel: w429 -> [w439 _]
          tunnel: w427 -> [w438 _]
          tunnel: [w437 w446] -> w426
          tunnel: w424 -> [w436 w446]
          frame False {
            n157 = call "SummaryWithGlyphManager.vi"("error in"=w440, "glyph manager"=w436, "node self ref"=w439) -> ("error out"=w442:errorcluster, "glyph manager out"=w435:T9, "summary"=w441:T16[])  [unwired: 6 in]
            n158 = call "RefreshSubTreeWithGlyphManager.vi"("error in"=w442, "glyph manager"=w435, "node information"=w441, "tree ref in"=w438) -> ("error out"=w445:errorcluster, "glyph manager out"=w437:T9, "tree ref out"=w443:refnum<vi>)  [unwired: 5 in]
            n159 = Close Reference(reference=w443, error in (no error)=w445) -> (error out=w444:errorcluster)
          }
          frame True {
          }
        }
        n160 = Bundle By Name(cluster=w425, "glyph manager"=w426) -> (w433:T1)
      }
      frame "RemoveNode" {
        n161 = call "IDtoNode.vi"("error in"=w455, "ID"=w456) -> ("error out"=w454:errorcluster, "invalid Id"=w451:bool, "node ref"=w453:T2)  [unwired: 7 in]
        n162 = case shown="False" w451 {
          tunnel: w454 -> [w463 w464]
          tunnel: w453 -> [w462 _]
          tunnel: [w459 w464] -> w452
          tunnel: w450 -> [w458 _]
          frame False {
            n163 = call "RemoveNode.vi"("error in"=w463, "node"=w462) -> ("error out"=w460:errorcluster, "node ID"=w461:string)  [unwired: 8 in]
            n164 = call "ClearTreeNode.vi"("error in"=w460, "tag"=w461, "tree reference"=w458) -> ("error out"=w459:errorcluster)  [unwired: 8 in]
          }
          frame True {
          }
        }
        n165 = Bundle By Name(cluster=w457, "unsaved changes"=TRUE) -> (w449:T1)
      }
      frame "PopulateTree" {
        n166 = Unbundle By Name(w486) -> ("current path"=w478:path, "standard events"=w469:T3, "glyph manager"=w466:T9, "root"=w482:T2)
        n167 = call "SummaryWithGlyphManager.vi"("error in"=w484, "glyph manager"=w466, "depth"=0 ("Depth"), "node self ref"=w482) -> ("error out"=w483:errorcluster, "glyph manager out"=w465:T9, "summary"=w485:T16[])  [unwired: 5 in]
        n168 = call <vilib>:"Check if File or Folder Exists.vi"("path"=w478) -> ("file or folder exists?"=w476:bool, "dup path"=w477:path)  [unwired: 8 in, 1 out]
        n169 = Strip Path(path=w477) -> (name=w475:string)  [unwired: 1 out]
        n170 = call "RefreshEntireTreeWithGlyphManager.vi"("calling VI in"=w472, "error in"=w483, "glyph manager"=w465, "array"=w485, "tree ref in"=w473) -> ("error out"=w480:errorcluster, "glyph manager out"=w467:T9)  [unwired: 5 in]
        n171 = Select(t=w475, s=w476, f="Advanced Configurator Sample Project") -> (s? t:f=w471:string)
        n172 = property class="VI"(reference=w472, "Front Panel.Title"=w471) -> ()  [unwired: 1 in, 2 out]
        n173 = call "ClearSubPanelStandardEvents.vi"("error in"=w480, "standard events"=w469, "sub panel ref in"=w470) -> ("error out"=w479:errorcluster)  [unwired: 7 in, 1 out]
        n174 = Bundle By Name(cluster=w486, "glyph manager"=w467) -> (w468:T1)
      }
      frame "CleansubPanel" {
        n175 = Unbundle By Name(w492) -> ("standard events"=w487:T3)
        n176 = call "ClearSubPanelStandardEvents.vi"("error in"=w493, "standard events"=w487, "sub panel ref in"=w488) -> ("error out"=w491:errorcluster, "sub panel ref out"=w490:refnum<vi>)  [unwired: 7 in]
        n177 = Close Reference(reference=w490, error in (no error)=w491) -> (error out=w489:errorcluster)
      }
      frame "ActivateNode" {
        n178 = Unbundle By Name(w497) -> ("standard events"=w496:T3)
        n179 = call "IDtoNode.vi"("error in"=w502, "ID"=w503) -> ("error out"=w495:errorcluster, "invalid Id"=w501:bool, "node ref"=w500:T2)  [unwired: 7 in]
        n180 = case shown="False" w501 {
          tunnel: w500 -> [w510 _]
          tunnel: [w511 w512] -> w499
          tunnel: w495 -> [w508 w512]
          tunnel: w498 -> [w507 _]
          tunnel: w496 -> [w504 _]
          tunnel: w494 -> [w505 _]
          frame False {
            n181 = call "ClearSubPanelStandardEvents.vi"("error in"=w508, "standard events"=w504, "sub panel ref in"=w505) -> ("error out"=w509:errorcluster, "sub panel ref out"=w506:refnum<vi>)  [unwired: 7 in]
            n182 = call "LoadNodeUIStandardEvents.vi"("user event out"=w504, "error in"=w509, "sub panel ref in"=w506, "main queue"=w507, "node"=w510) -> ("error out"=w511:errorcluster)  [unwired: 6 in]
          }
          frame True {
          }
        }
      }
      frame "Move" {
        n183 = Unflatten From String(type=T13 {"node ref"=refnum, "new parent"=refnum, "Index"=0} ("Cluster"), binary string=w526, error in (no error)=w524) -> (value=w523:T13, error out=w522:errorcluster)  [unwired: 2 in, 1 out]
        n184 = Unbundle By Name(w523) -> ("node ref"=w517:T2, "new parent"=w516:T2, "Index"=w513:i32)
        n185 = call "MoveNode.vi"("error in"=w522, "index"=w513, "new parent"=w516, "node"=w517) -> ("error out"=w520:errorcluster)  [unwired: 7 in]
        n186 = Bundle By Name(cluster=w527, "unsaved changes"=TRUE) -> (w515:T1)
        n187 = call <vilib>:"Send Local Message.vi"("message queue in"=w518, "message name"="PopulateTree", "error in"=w520) -> ("error out"=w519:errorcluster)  [unwired: 10 in, 2 out]
      }
      frame "NodeDataChange" {
        n188 = call <vilib>:"Send Local Message.vi"("message queue in"=w528, "message name"="RefreshNode", "message value"=w529, "error in"=w531) -> ("error out"=w530:errorcluster)  [unwired: 9 in, 2 out]
        n189 = Bundle By Name(cluster=w535, "unsaved changes"=TRUE) -> (w534:T1)
      }
    }
  }
  n190 = while "User Interface Event Handler" {
    tunnel: w17 -> [w542]
    tunnel: w8 -> [w538]
    tunnel: w5 -> [w537]
    tunnel: [w536] -> w6
    stop <- w541 stop-if-true
    n191 = event shown="[2] \"View\": Drop" {
      selector: w537 -> [_ _ _ _ _ _ _ _ _ _]
      dyn-events: [_ _ _ _ _ _ _ _ _ _] -> w536
      timeout: _ -> [_ _ _ _ _ _ _ _ _ _]
      tunnel: w542 -> [w551 w576 w626 w655 w662 w691 w696 w706 w712 w756]
      tunnel: [_ _ _ TRUE _ _ _ _ _ _] -> w541
      tunnel: [w551 w573 w624 w651 w662 w688 w696 w704 w711 w755] -> w540
      tunnel: [w547 w572 w623 w652 w658 w687 w693 w702 w709 _] -> w539
      tunnel: w538 -> [w550 w571 w625 w653 w661 w686 w695 w703 w710 _]
      event "View": Shortcut Menu Activation? {
        n192 = event-data() -> ("CtlRef"=w557:refnum<vi>, "Coords"=w556:T17, "MenuRef"=w553:refnum<k9>)  [unwired: 1 in]
        n193 = invoke class="Tree (strict)" method="Point To Row Column"(reference=w557, error in=w550, "Point"=w556) -> (error out=w549:errorcluster, "Tag"=w555:string)  [unwired: 5 in, 6 out]
        n194 = call "IDtoNode.vi"("error in"=w549, "ID"=w555) -> ("error out"=w545:errorcluster, "invalid Id"=w552:bool, "node ref"=w554:T2)  [unwired: 7 in]
        n195 = case shown="False" w552 {
          selector: w552 -> [_ w568]
          tunnel: w554 -> [w562 _]
          tunnel: w553 -> [w561 _]
          tunnel: [w560 _] -> w548
          tunnel: [w559 _] -> w546
          tunnel: w545 -> [w558 w569]
          tunnel: [w558 w569] -> w544
          tunnel: [_ w568] -> w543
          frame False {
            n196 = in-place {
              in-place-border: w561 -> [w565]
              in-place-border: [w563] -> w560
              n197 = in-place-dvr #7(w562) -> (w567:refnum<class "NISE_CEF_Node.lvclass">, w564:errorcluster)
              n198 = call-dynamic "ShortcutMenu.vi"("error in"=w564, "menu ref in"=w565, "node in"=w567) -> ("error out"=w563:errorcluster, "node out"=w566:refnum<class "NISE_CEF_Node.lvclass">)  [unwired: 6 in, 1 out]
              n199 = in-place-dvr #7(w566) -> (w559:errorcluster)  [unwired: 1 out]
            }
          }
          frame True {
          }
        }
        n200 = Merge Errors(w546, w548, w544) -> (w547:errorcluster)
        n201 = event-data("Discard?"=w543) -> ()  [unwired: 1 in, 1 out]
      }
      event "View": Shortcut Menu Selection (User) {
        n202 = event-data() -> ("ItemPath"=w575:string, "CtlRef"=w579:refnum<vi>, "Coords"=w580:T17)  [unwired: 1 in]
        n203 = invoke class="Tree (strict)" method="Point To Row Column"(reference=w579, error in=w571, "Point"=w580) -> (error out=w570:errorcluster, "Tag"=w574:string)  [unwired: 5 in, 6 out]
        n204 = Match Pattern(string=w575, regular expression=":") -> (before substring=w578:string, after substring=w577:string)  [unwired: 1 in, 2 out]
        n205 = case shown="Default" w578 {
          selector: w578 -> [w582 _ _ _]
          tunnel: w577 -> [_ _ _ w607]
          tunnel: w576 -> [w589 w596 w602 w609]
          tunnel: w574 -> [w584 w594 w600 w608]
          tunnel: [w586 w593 w599 w605] -> w573
          tunnel: [w587 w592 w597 w603] -> w572
          tunnel: w570 -> [w588 w591 w598 w604]
          frame Default {
            n206 = Concatenate Strings(w582, ":" ("string"), w584) -> (w585:string)
            n207 = call <vilib>:"Send Local Message.vi"("message queue in"=w589, "message name"="CustomMenuAction" ("Message Name"), "message value"=w585, "error in"=w588) -> ("message queue out"=w586:T11, "error out"=w587:errorcluster)  [unwired: 9 in, 1 out]
          }
          frame "Remove" {
            n208 = call <vilib>:"Send Local Message.vi"("message queue in"=w596, "message name"="RemoveNode" ("Message Name"), "message value"=w594, "error in"=w591) -> ("message queue out"=w593:T11, "error out"=w592:errorcluster)  [unwired: 9 in, 1 out]
          }
          frame "Duplicate" {
            n209 = call <vilib>:"Send Local Message.vi"("message queue in"=w602, "message name"="Duplicate" ("Message Name"), "message value"=w600, "error in"=w598) -> ("message queue out"=w599:T11, "error out"=w597:errorcluster)  [unwired: 9 in, 1 out]
          }
          frame "Add" {
            n210 = Bundle By Name(cluster=T12 {"node type"="", "to add to"=""} ("input cluster"), "node type"=w607, "to add to"=w608) -> (w610:T12)
            n211 = Flatten To String(anything=w610) -> (data string=w611:string)  [unwired: 3 in, 2 out]
            n212 = call <vilib>:"Send Local Message.vi"("message queue in"=w609, "message name"="AddNode" ("Message Name"), "message value"=w611, "error in"=w604) -> ("message queue out"=w605:T11, "error out"=w603:errorcluster)  [unwired: 9 in, 1 out]
          }
        }
      }
      event "View": Drop {
        n213 = event-data() -> ("CtlRef"=w629:refnum<vi>, "Coords"=w628:T17)  [unwired: 1 in]
        n214 = invoke class="Tree (strict)" method="Point To Row Column"(reference=w629, error in=w625, "Point"=w628) -> (reference out=w627:refnum<vi>, error out=w622:errorcluster, "Tag"=w620:string)  [unwired: 5 in, 5 out]
        n215 = call "ValidDragDrop.vi"("error in"=w622, "Reorder"=TRUE, "drag over"=w620, "Tree Ref in"=w627) -> ("Error Out"=w616:errorcluster, "Accepted"=w618:bool, "Drag"=w621:string, "Tree Ref out"=w631:refnum<vi>, "Moved Node"=w617:T2, "Position"=w615:i32, "Parent Node"=w619:T2, "Parent"=w614:string)
        n216 = case shown="False" w618 {
          tunnel: w621 -> [_ w648]
          tunnel: w631 -> [_ w650]
          tunnel: [_ TRUE] -> w630
          tunnel: w614 -> [_ w646]
          tunnel: w626 -> [w633 w645]
          tunnel: [w633 w641] -> w624
          tunnel: [w632 w640] -> w623
          tunnel: w617 -> [_ w637]
          tunnel: w619 -> [_ w635]
          tunnel: w616 -> [w632 w636]
          tunnel: w615 -> [_ w634]
          frame False {
          }
          frame True {
            n217 = invoke class="Tree (strict)" method="Edit Tree Items.Move Item"(reference=w650, error in=w636, "tag"=w648, "New Parent"=w646) -> (error out=w638:errorcluster)  [unwired: 3 in, 6 out]
            n218 = Bundle By Name(cluster=T13 {"node ref"=refnum, "new parent"=refnum, "Index"=0} ("Cluster"), "Index"=w634, "node ref"=w637, "new parent"=w635) -> (w644:T13)
            n219 = Flatten To String(anything=w644, error in (no error)=w638) -> (data string=w643:string, error out=w639:errorcluster)  [unwired: 2 in, 1 out]
            n220 = call <vilib>:"Send Local Message.vi"("message queue in"=w645, "message name"="Move", "message value"=w643, "error in"=w639) -> ("message queue out"=w641:T11, "error out"=w640:errorcluster)  [unwired: 9 in, 1 out]
          }
        }
        n221 = event-data("Accepted?"=w630) -> ()  [unwired: 1 in, 1 out]
      }
      event "Exit": Value Change {
        # "Exit the application                                           >> Stop this message generator loop    Cleaning errors if the other loop stop this one"
        n222 = event-data() -> ()  [unwired: 1 in, 1 out]
        n223 = call <vilib>:"Send Local Message.vi"("message queue in"=w655, "message name"="Close", "error in"=w653) -> ("message queue out"=w651:T11, "error out"=w656:errorcluster)  [unwired: 10 in, 1 out]
        n224 = call <vilib>:"Clear Errors.vi"("error in (no error)"=w656) -> ("error out"=w652:errorcluster)  [unwired: 5 in, 1 out]
      }
      event "View": Drag Starting? {
        n225 = event-data() -> ("Data"=w668:T18, "CtlRef"=w670:refnum<vi>, "Coords"=w669:T17)  [unwired: 1 in]
        n226 = invoke class="Tree (strict)" method="Point To Row Column"(reference=w670, error in=w661, "Point"=w669) -> (error out=w660:errorcluster, "Tag"=w667:string)  [unwired: 5 in, 6 out]
        n227 = call "IDtoNode.vi"("error in"=w660, "ID"=w667) -> ("error out"=w659:errorcluster, "invalid Id"=w666:bool, "node ref"=w665:T2)  [unwired: 7 in]
        n228 = case shown="False" w666 {
          tunnel: w665 -> [w678 _]
          tunnel: [w675 TRUE ("Removable")] -> w663
          tunnel: w659 -> [w674 w684]
          tunnel: [w671 w684] -> w658
          frame False {
            n229 = in-place {
              in-place-border: [w681] -> w677
              in-place-border: w674 -> [w680]
              in-place-border: [w679] -> w673
              n230 = in-place-dvr #8(w678) -> (w683:refnum<class "NISE_CEF_Node.lvclass">)  [unwired: 1 out]
              n231 = call-dynamic "EditOptions.vi"("error in"=w680, "node in"=w683) -> ("error out"=w679:errorcluster, "edit options"=w681:T19, "node out"=w682:refnum<class "NISE_CEF_Node.lvclass">)  [unwired: 6 in, 1 out]
              n232 = in-place-dvr #8(w682) -> (w672:errorcluster)  [unwired: 1 out]
            }
            n233 = Unbundle By Name(w677) -> ("movable"=w676:bool)
            n234 = Merge Errors(w672, w673) -> (w671:errorcluster)
            n235 = Not(x=w676) -> (.not. x?=w675:bool)
          }
          frame True {
          }
        }
        n236 = event-data("Data"=w668, "Drag Mode"=enum32{"copy or move", "copy only", "move only"}."move only", "Discard?"=w663) -> ()  [unwired: 1 in, 1 out]
      }
      event "View": Value Change {
        n237 = event-data() -> ("NewVal"=w689:string)  [unwired: 1 in]
        n238 = call <vilib>:"Send Local Message.vi"("message queue in"=w691, "message name"="ActivateNode" ("Message Name"), "message value"=w689, "error in"=w686) -> ("message queue out"=w688:T11, "error out"=w687:errorcluster)  [unwired: 9 in, 1 out]
      }
      event "View": event type 3.0.xa000003a {
        n239 = event-data() -> ("CtlRef"=w701:refnum<vi>, "Coords"=w698:T17)  [unwired: 1 in]
        n240 = invoke class="Tree (strict)" method="Point To Row Column"(reference=w701, error in=w695, "Point"=w698) -> (reference out=w700:refnum<vi>, error out=w694:errorcluster, "Tag"=w699:string)  [unwired: 5 in, 5 out]
        n241 = call "ValidDragDrop.vi"("error in"=w694, "Reorder"=TRUE, "drag over"=w699, "Tree Ref in"=w700) -> ("Error Out"=w693:errorcluster, "Accepted"=w697:bool)  [unwired: 6 out]
        n242 = event-data("Accepted?"=w697) -> ()  [unwired: 1 in, 1 out]
      }
      event Panel Close? {
        # "Intercepts the upper right close panel operation to allow a smooth shutdown as opposed to immediately killing the app."
        n243 = event-data() -> ()  [unwired: 1 in, 1 out]
        n244 = call <vilib>:"Send Local Message.vi"("message queue in"=w706, "message name"="Close?", "error in"=w703) -> ("message queue out"=w704:T11, "error out"=w702:errorcluster)  [unwired: 10 in, 1 out]
        n245 = event-data("Discard?"=TRUE) -> ()  [unwired: 1 in, 1 out]
      }
      event Menu Selection (User) {
        # "#USERCFG It is needed to add a Case for Every item on the menu"
        n246 = event-data() -> ("ItemTag"=w708:string, "ItemPath"=w713:string)  [unwired: 1 in]
        n247 = case shown="\"_File:_New\"" w713 {
          selector: w713 -> [_ _ _ _ _ w743]
          tunnel: w712 -> [w718 w723 w728 w733 w738 w751]
          tunnel: [w714 w719 w724 w729 w734 w748] -> w711
          tunnel: w710 -> [w716 w721 w726 w731 w736 w739]
          tunnel: [w715 w720 w725 w730 w735 w746] -> w709
          tunnel: w708 -> [_ _ _ _ _ w744]
          frame "_File:_New" {
            n248 = call <vilib>:"Send Local Message.vi"("message queue in"=w718, "message name"="New?" ("Message Name"), "error in"=w716) -> ("message queue out"=w714:T11, "error out"=w715:errorcluster)  [unwired: 10 in, 1 out]
          }
          frame "_File:_Open" {
            n249 = call <vilib>:"Send Local Message.vi"("message queue in"=w723, "message name"="Open?" ("Message Name"), "error in"=w721) -> ("message queue out"=w719:T11, "error out"=w720:errorcluster)  [unwired: 10 in, 1 out]
          }
          frame "_File:_Save" {
            n250 = call <vilib>:"Send Local Message.vi"("message queue in"=w728, "message name"="Save" ("Message Name"), "error in"=w726) -> ("message queue out"=w724:T11, "error out"=w725:errorcluster)  [unwired: 10 in, 1 out]
          }
          frame "_File:Save As..." {
            n251 = call <vilib>:"Send Local Message.vi"("message queue in"=w733, "message name"="SaveAs" ("Message Name"), "error in"=w731) -> ("message queue out"=w729:T11, "error out"=w730:errorcluster)  [unwired: 10 in, 1 out]
          }
          frame "_File:_Exit" {
            n252 = call <vilib>:"Send Local Message.vi"("message queue in"=w738, "message name"="Close?" ("Message Name"), "error in"=w736) -> ("message queue out"=w734:T11, "error out"=w735:errorcluster)  [unwired: 10 in, 1 out]
          }
          frame Default {
            n253 = Bundle("ItemTag"=w744, w743) -> (w742:cluster{"ItemTag":string, string})  [unwired: 1 in]
            n254 = Flatten To String(anything=w742, error in (no error)=w739) -> (data string=w741:string, error out=w740:errorcluster)  [unwired: 2 in, 1 out]
            n255 = call <vilib>:"Send Local Message.vi"("message queue in"=w751, "message name"="CleansubPanel", "error in"=w740) -> ("message queue out"=w750:T11, "error out"=w747:errorcluster)  [unwired: 10 in, 1 out]
            n256 = call <vilib>:"Send Local Message.vi"("message queue in"=w750, "message name"="CustomFileMenu" ("Message Name"), "message value"=w741, "error in"=w747) -> ("message queue out"=w748:T11, "error out"=w746:errorcluster)  [unwired: 9 in, 1 out]
          }
        }
      }
      event User Event {
        n257 = event-data() -> ("node ref"=w754:T2)  [unwired: 1 in]
        n258 = call "NodetoID.vi"("node ref"=w754) -> ("ID"=w752:string)  [unwired: 9 in, 1 out]
        n259 = call <vilib>:"Send Local Message.vi"("message queue in"=w756, "message name"="NodeDataChange", "message value"=w752) -> ("message queue out"=w755:T11)  [unwired: 10 in, 2 out]
      }
    }
    n260 = call "Error.vi"("error in (no error)"=w539, "message queue in"=w540) -> ()  [unwired: 9 in, 1 out]
  }
  n261 = Unregister For Events(event registration refnum=w6) -> (error out=w2:errorcluster)  [unwired: 1 in]
  n262 = Merge Errors(w2, w1) -> (w3:errorcluster)
  n263 = call "DestroyStandardEvents.vi"("error in"=w3, "standard events"=w4) -> ()  [unwired: 9 in, 1 out]
